vi "FuncVI-UWNoise.vi"(5 "InstanceRef":T2, 9 "arg list":T1[](array[typedef]) {"num" format="%.2f"}) -> (0 "error out":bool, 3 "result":T1 {"num" format="%.2f"})   [LabVIEW 2021]
doc: "::: CalcExpress Toolkit :::\nCopyright (c) 2000-2026 Konstantin Shifershteyn. All rights reserved."
uses:
  cetypes.llb/CalcExpress Function Argument Info.ctl
  cetypes.llb/CalcExpress Instance RefNum.ctl
  <vilib>/Analysis/NI_AALBase.lvlib
panel:
  in  "max arg num":i32=3
  in  "min arg num":i32
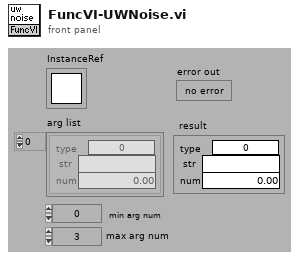
[diagram p1: front panel]
types:
  T1 = typedef "CalcExpress Function Argument Info.ctl" = cluster{"type":u32, "str":string, "num":dbl}
  T2 = typedef "CalcExpress Instance RefNum.ctl" = refnum<k1>
  T3 = enum8{"String", "DBL Number", "identifier", "1D Array of DBL", "2D Array of DBL", "CDB Number", "1D Array of CDB", "2D Array of CDB", "1D Array of String", "2D Array of String", "Unknown data type"}
  T4 = cluster{"index":i32, "type":enum8{"String", "DBL Number", "identifier", "1D Array of DBL", "2D Array of DBL", "CDB Number", "1D Array of CDB", "2D Array of CDB", "Unknown data type"}, "default num":dbl, "default str":string}[]
  T5 = cluster{"num list[0]":dbl, "num list[1]":dbl, "num list[2]":dbl}
  T6 = cluster{"type":enum8{"String", "DBL Number", "identifier", "1D Array of DBL", "2D Array of DBL", "CDB Number", "1D Array of CDB", "2D Array of CDB", "1D Array of String", "2D Array of String", "Unknown data type"}, "data string":string, dbl}
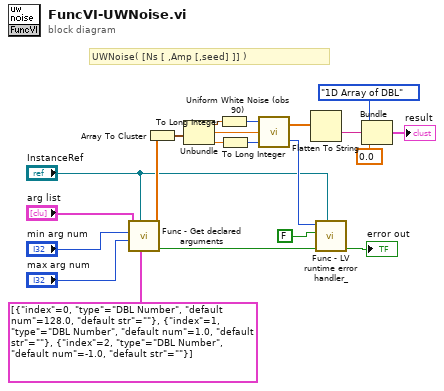
[diagram p0: block diagram]
diagram:
  # "UWNoise( [Ns [ ,Amp [,seed] ]] )"
  n1 = call "Func - Get declared arguments.vi"("arg descriptors"=T4 [{"index"=0, "type"=enum."DBL Number", "default num"=128.0, "default str"=""}, {"index"=1, "type"=enum."DBL Number", "default num"=1.0, "default str"=""}, {"index"=2, "type"=enum."DBL Number", "default num"=-1.0, "default str"=""}] ("args descriptors"), "InstanceRef"="InstanceRef", "max arg num"="max arg num", "min arg num"="min arg num", "arg list"="arg list") -> ("error out"=w11:bool, "num list"=w20:dbl[])  [unwired: 3 in, 2 out]
  n2 = Array To Cluster(array=w20) -> (cluster=w18:T5)
  n3 = Unbundle(w18) -> ("num list[0]"=w13:dbl, "num list[1]"=w14:dbl, "num list[2]"=w6:dbl)
  n4 = To Long Integer(number=w13) -> (32bit integer=w12:i32)
  n5 = To Long Integer(number=w6) -> (32bit integer=w5:i32)
  n6 = call <vilib>:"Uniform White Noise (obs 90).vi"("seed"=w5, "amplitude"=w14, "samples"=w12) -> ("error"=w10:i32, "uniform white noise"=w8:dbl[])
  n7 = Flatten To String(anything=w8) -> (data string=w7:string)  [unwired: 3 in, 2 out]
  n8 = call "Func - LV runtime error handler_.vi"("InstanceRef"="InstanceRef", "error in"=w11, "Gen CE error?"=FALSE, "LabVIEW error code"=w10) -> ("error out"=→"error out":bool)  [unwired: 7 in]
  n9 = Bundle("type"=T3."1D Array of DBL", "data string"=w7, 0.0) -> (→"result":T6)  [unwired: 1 in]
